vi "SMTP Email Send File.vi"(0 "recipients":string[](array[string]) caption="destinataires", 1 "mail server":string caption="serveur mail", 2 "return address":string caption="adresse de retour", 5 "subject ([No Subject])":string="[Sans objet]" caption="objet ([Sans objet])", 7 "message":string, 9 "file path":path caption="chemin du fichier", 11 "error in (no error)":errorcluster caption="entrée d'erreur (pas d'erreur)", 12 "binary? (F)":bool caption="binaire ? (F)", 13 "MIME content-type (application/octet-stream)":string="application/octet-stream" caption="type de contenu MIME (application/octet-stream)") -> (4 "invalid recipients":string[](array[string]) caption="destinataires non valides", 15 "error out":errorcluster caption="sortie d'erreur")   [LabVIEW 2022 SP3, in "Copie de NI_SMTPEmail.lvlib"]
doc: "LabVIEW ne supporte plus ce VI. À la place, utilisez le VI Express Envoyer un e-mail.\n\nEnvoie un e-mail avec un fichier en pièce jointe à une liste de destinataires.\n\n<b>adresse de retour</b> est l'adresse-email de l'expéditeur du message. Si vous ne spécifiez pas d'adresse de retour, une chaîne vide est envoyée au serveur. Vous n'êtes pas obligé d'inclure une adresse de retour pour que ce VI fonctionne, mais certains serveurs de messagerie n'acceptent pas les messages si ces informations sont absentes. \n<b>serveur mail</b> est le nom ou l'adresse IP d'un serveur SMTP valide. Si vous passez une chaîne vide à cette entrée, LabVIEW n'accepte pas la connexion réseau et renvoie l'erreur 63. \n<b>destinataires</b> est le tableau de chaînes qui contient les adresses e-mail des destinataires du message. Chaque adresse peut être un élément de tableau séparé. \n<b>objet</b> est la ligne d'objet du message. La valeur par défaut est [Sans objet]. \n<b>message</b> correspond au message textuel de l'e-mail, formaté avec le jeu de caractères système. LabVIEW convertit cette chaîne en format UTF-8 avant d'envoyer l'e-mail. \n<b>chemin de fichier</b> est le chemin vers le fichier que vous voulez mettre en pièce jointe. Vous pouvez lier une chaîne ou un fichier de l'ordinateur local. \n<b>entrée d'erreur</b> décrit les conditions d'erreur qui ont lieu avant l'exécution de ce nœud. Cette entrée fournit la fonctionnalité d'entrée d'erreur standard. \n<b>binaire ?</b> spécifie si la pièce jointe est au format texte, décrite par le paramètre <b>jeu de caractères</b>, ou binaire, décrite par le paramètre <b>type de contenu MIME</b>. La valeur par défaut est FAUX, ce qui spécifie une pièce jointe de type texte.\n<b>type de contenu MIME</b> détermine le type de contenu pour une pièce jointe de type binaire. Vous pouvez spécifier n'importe quel type de contenu supporté par la norme RFC 2045, y compris les types de contenu courants suivants :\n\napplication/octet-stream (valeur par défaut) : indique un fichier binaire générique.\n\nimage/jpeg : indique des images JPEG.\n\ntext/html : indique des documents au format HTML.\n\n<b>destinataires non valides</b> liste les destinataires rejetés par le serveur mail. \n<b>sortie d'erreur</b> contient des informations sur l'erreur. Cette sortie fournit la fonctionnalité de sortie d'erreur standard."
uses:
  Copie de NI_SMTPEmail.lvlib
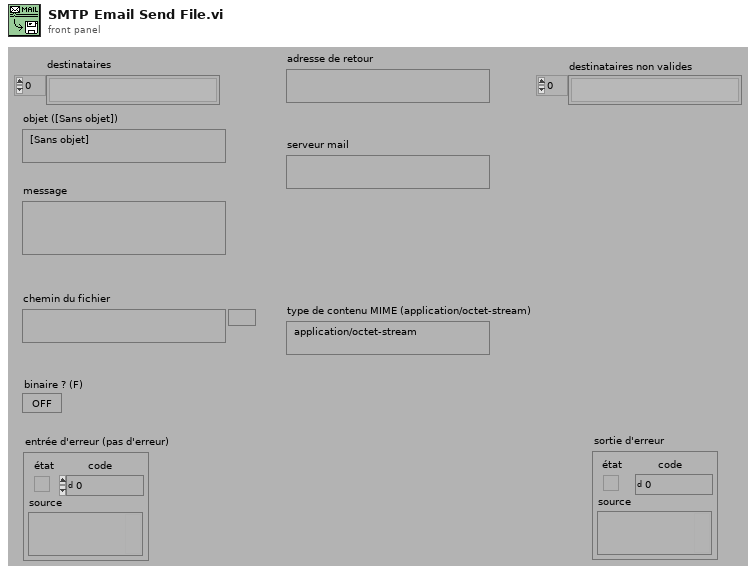
[diagram p1: front panel]
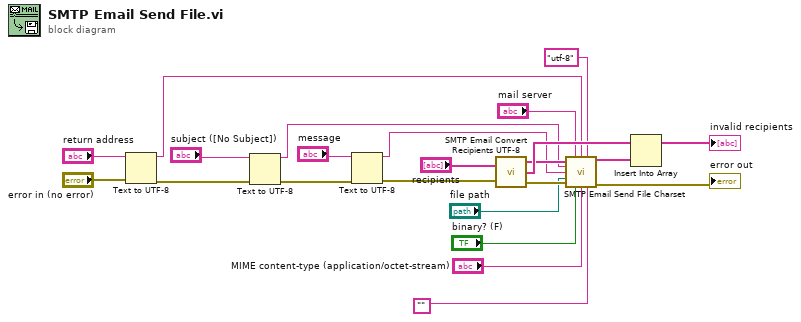
[diagram p0: block diagram]
diagram:
  n1 = Text to UTF-8(8:"error in (no error)", 11:"return address") -> (0:w18:errorcluster, 3:w8:string)  [unwired: 1 in]
  n2 = Text to UTF-8(8:w18, 11:"subject ([No Subject])") -> (0:w20:errorcluster, 3:w6:string)  [unwired: 1 in]
  n3 = Text to UTF-8(8:w20, 11:"message") -> (0:w22:errorcluster, 3:w5:string)  [unwired: 1 in]
  n4 = call "SMTP Email Convert Recipients UTF-8.vi"("recipients"="recipients", "error in"=w22) -> ("convertible recipients"=w10:string[], "unconvertible recipients"=w12:string[], "error out"=w15:errorcluster)
  n5 = call "SMTP Email Send File Charset.vi"("recipients"=w10, "mail server"="mail server", "return address"=w8, "character set (us-ascii)"="utf-8", "subject ([No Subject])"=w6, "message"=w5, "file path"="file path", "error in (no error)"=w15, "binary? (F)"="binary? (F)", "MIME content-type (application/octet-stream)"="MIME content-type (application/octet-stream)", "translit"="") -> ("invalid recipients"=w16:string[], "error out"=→"error out":errorcluster)  [unwired: 3 in]
  n6 = Insert Into Array(array=w12, new element=w16) -> (→"invalid recipients":string[])  [unwired: 1 in]
